vi "Disk_Check.vi"(7 "limit":dbl, 8 "error in":errorcluster, 10 "current File":path, 11 "path":path) -> (0 "error out":errorcluster)   [LabVIEW 2025]
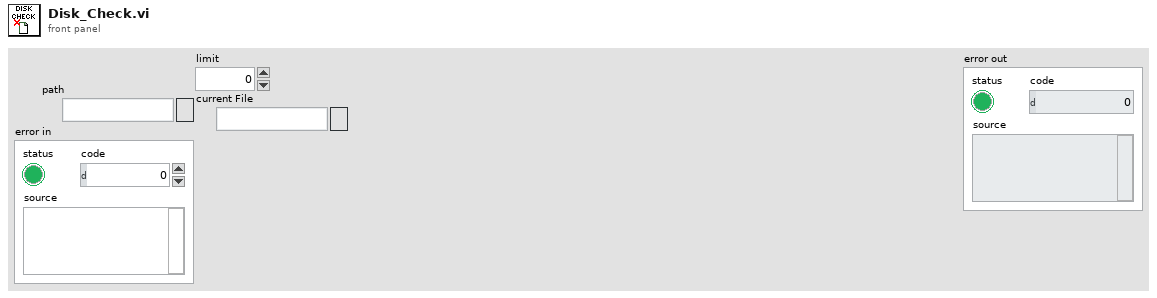
[diagram p1: front panel]
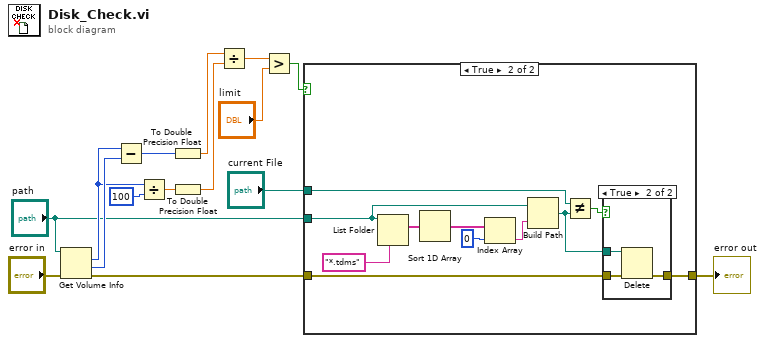
[diagram p0: block diagram]
diagram:
  n1 = Get Volume Info(8:"error in", 11:"path") -> (0:w2:errorcluster, 1:w14:i64, 2:w13:i64)  [unwired: 3 out]
  n2 = Subtract(x=w13, y=w14) -> (x-y=w9:i64)
  n3 = Divide(x=w13, y=i64 100) -> (x/y=w7:dbl)
  n4 = To Double Precision Float(number=w9) -> (double precision float=w8:dbl)
  n5 = To Double Precision Float(number=w7) -> (double precision float=w6:dbl)
  n6 = Divide(x=w8, y=w6) -> (x/y=w11:dbl)
  n7 = Greater?(x=w11, y="limit") -> (0:w5:bool)
  n8 = case shown="True" w5 {
    tunnel: "current File" -> [_ w21]
    tunnel: "path" -> [_ w22]
    tunnel: w2 -> [w16 w18]
    tunnel: [w16 w17] -> w1
    frame False {
    }
    frame True {
      n9 = List Folder(path=w22, pattern="*.tdms") -> (filenames=w26:string[])  [unwired: 2 in, 3 out]
      n10 = Sort 1D Array(array=w26) -> (sorted array=w25:string[])
      n11 = Index Array(array=w25, index=0) -> (element=w23:string)
      n12 = Build Path(base path=w22, name or relative path=w23) -> (appended path=w19:path)
      n13 = Not Equal?(x=w21, y=w19) -> (x != y?=w20:bool)
      n14 = case shown="True" w20 {
        tunnel: w19 -> [_ w31]
        tunnel: w18 -> [w28 w30]
        tunnel: [w28 w29] -> w17
        frame False {
        }
        frame True {
          n15 = Delete(path (use dialog)=w31, error in=w30) -> (error out=w29:errorcluster)  [unwired: 3 in, 2 out]
        }
      }
    }
  }
  "error out" <- w1
